vi "BigMAQ.vi"() -> ()   [LabVIEW 2019]
panel:
  out "Array 7":dbl[](array[numeric])
  out "Array 6":dbl[](array[numeric])
  out "Array 5":dbl[](array[numeric])
  out "Array 4":dbl[](array[numeric])
  out "Array 3":dbl[](array[numeric])
  out "Array 2":dbl[](array[numeric])
  out "x+y 2":dbl[](array[numeric])
  out "x+y":dbl[](array[numeric])
  out "Array":bool[](array[boolean])
  in  "IDs":T1
  out "Names":string[](array[string])
  in  "Status State":string="UI: Status"
  in  "Status":string
  out "States Out 2":string
  out "States Out":string
  out "Current State 2":string
  out "Arguments":string
  out "Current State":string
  out "Numeric 2":dbl
  out "Numeric":dbl
  in  "Image Data Range":cluster{dbl, dbl}(slide)={100.0, 0.0} scale=0.0..100.0
  out "SVG Object":T2
  in  "Name":string
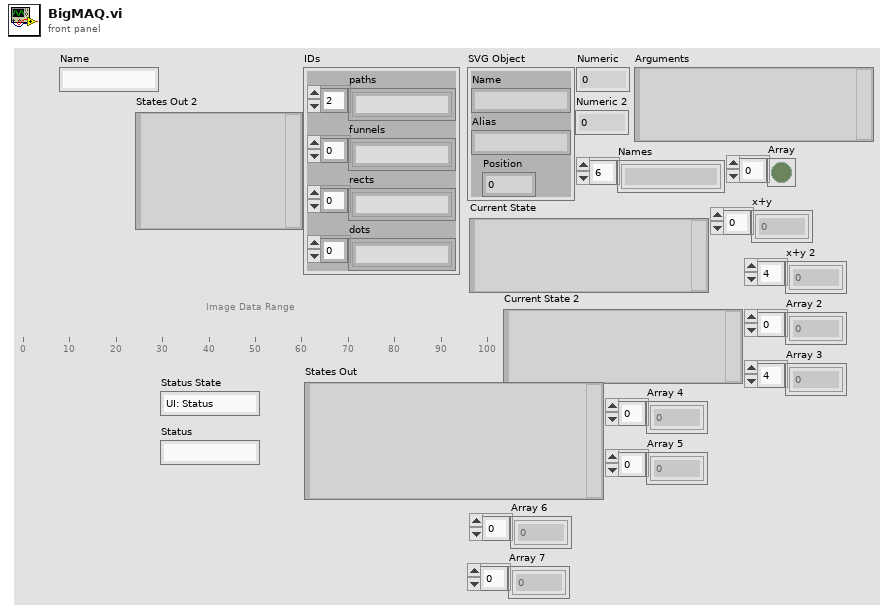
[diagram p1: front panel]
types:
  T1 = cluster{"paths":string[], "funnels":string[], "rects":string[], "dots":string[]}
  T2 = cluster{"Name":string, "Alias":string, "Position":i32}
  T3 = cluster{"Name":string, "Alias":string, "Position":i32}[]
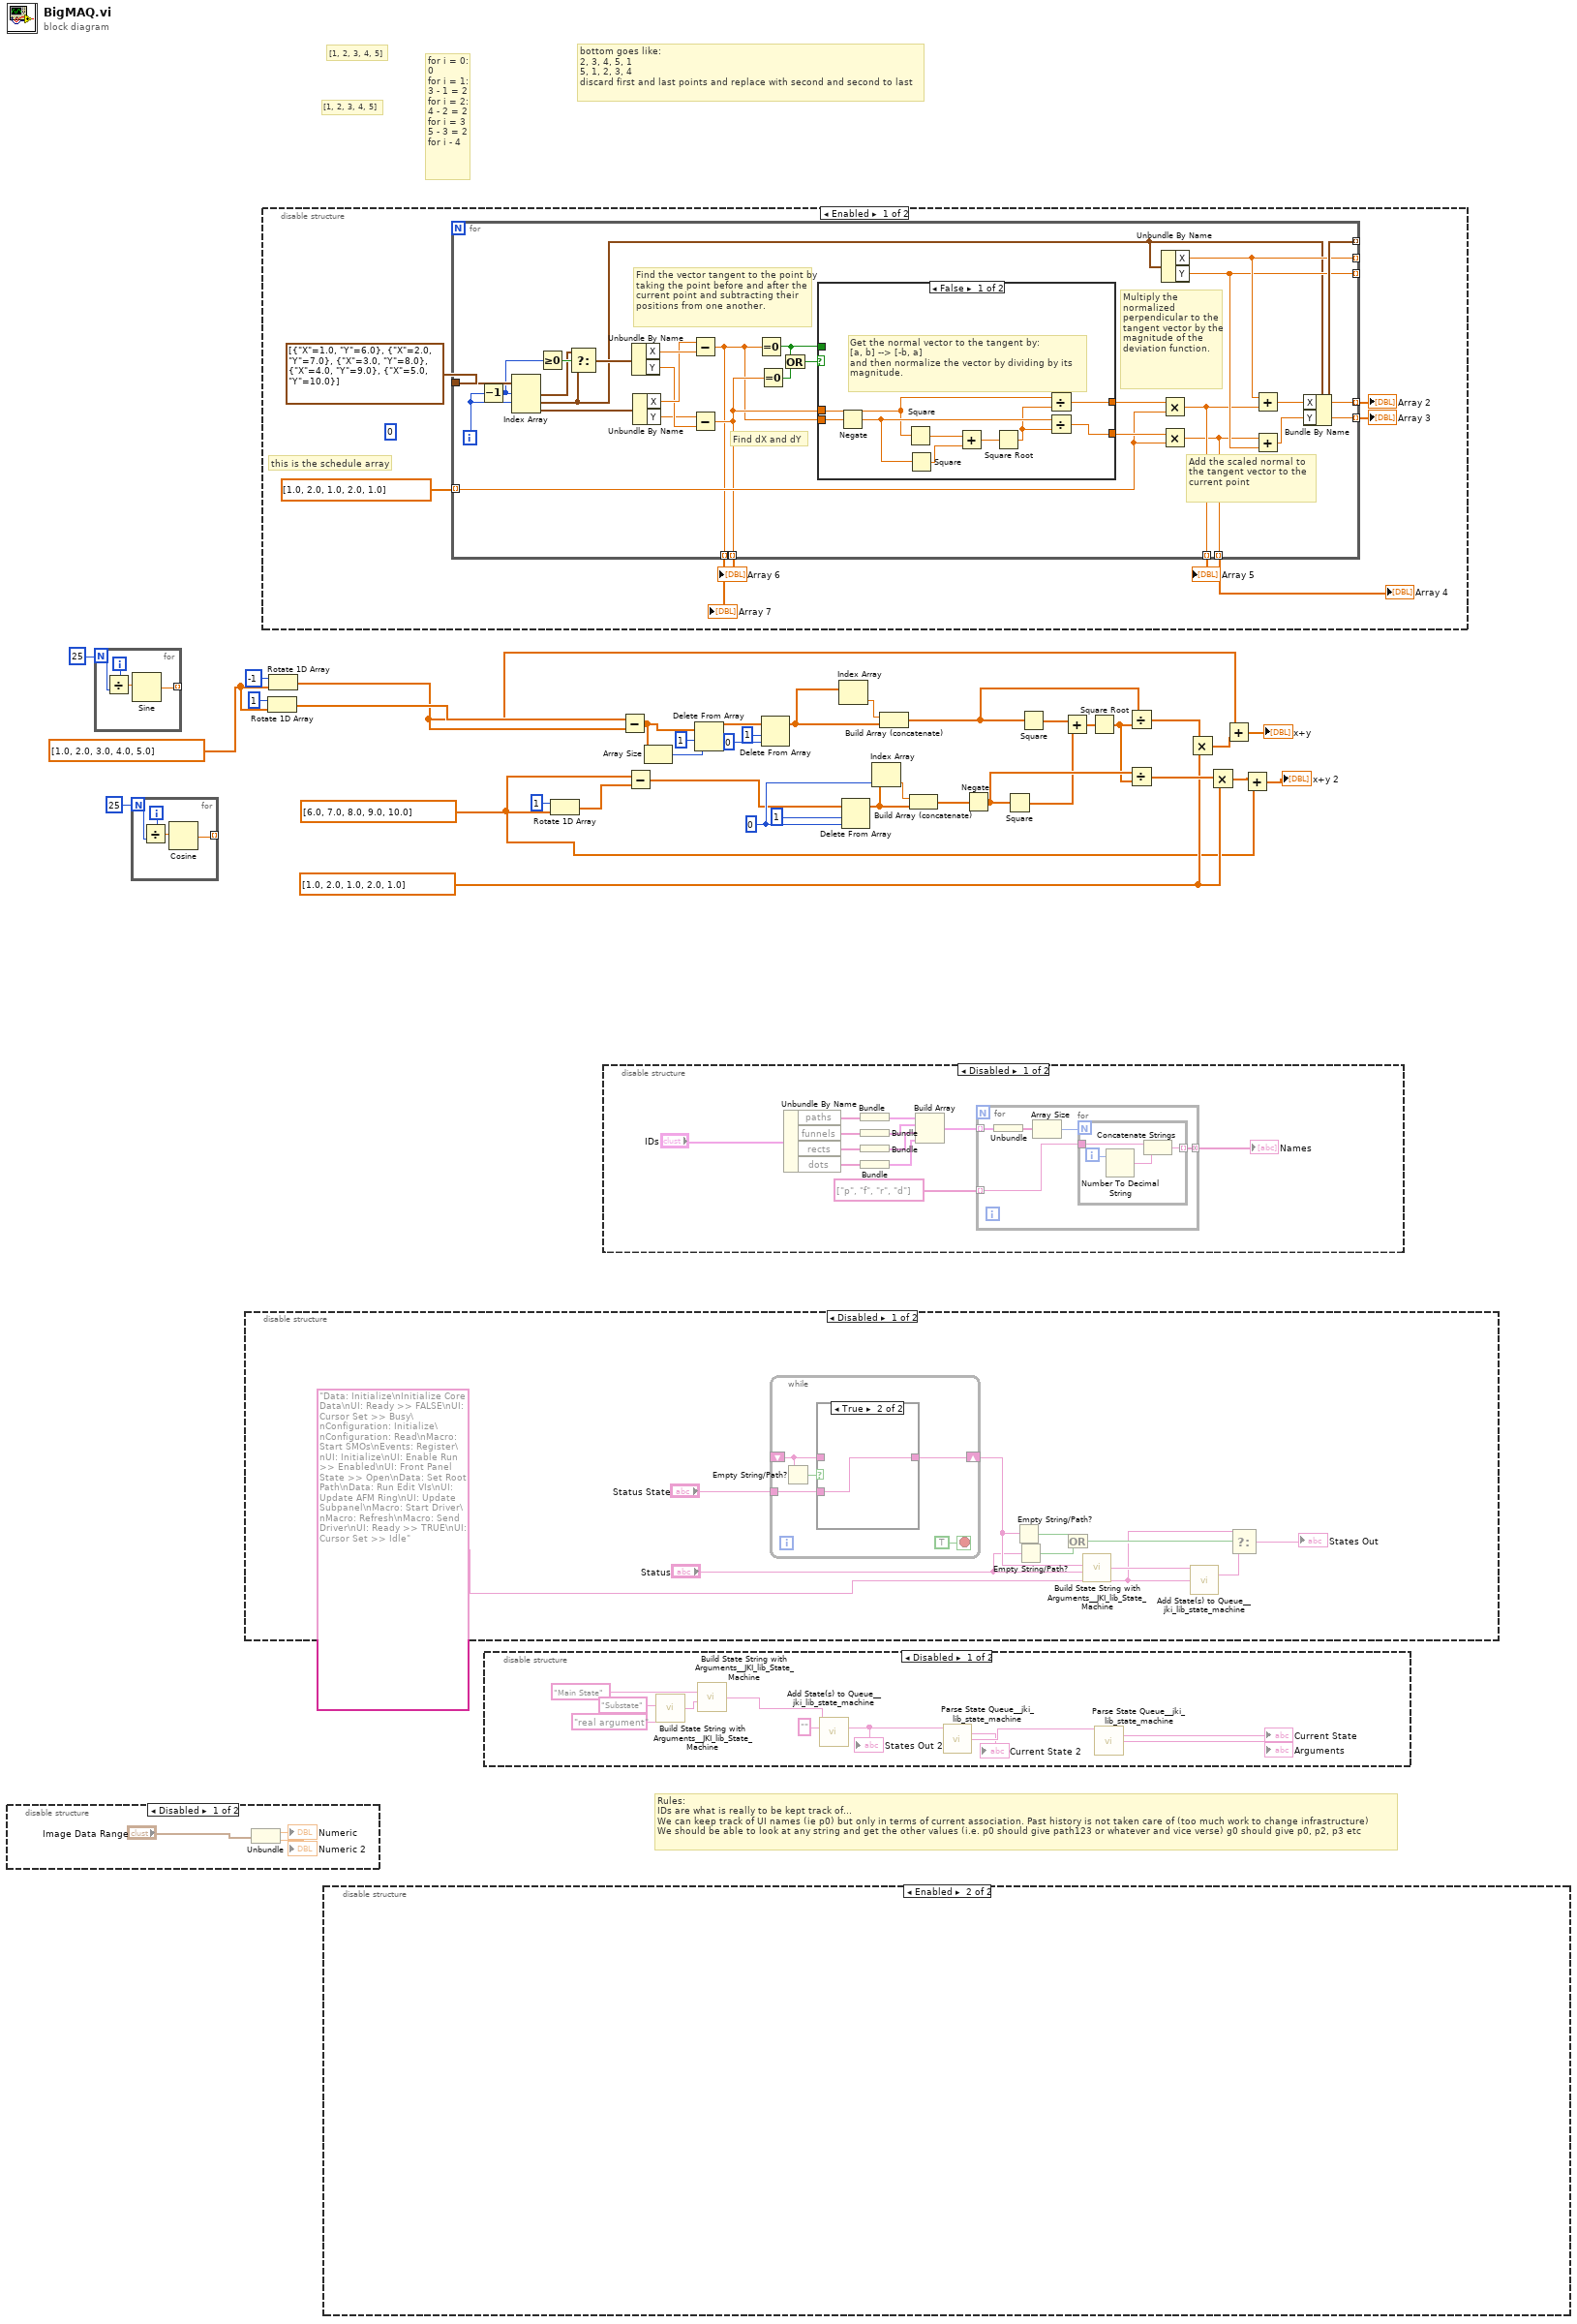
[diagram p0: block diagram]
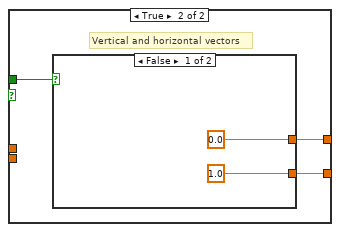
[diagram p7: hidden frame]
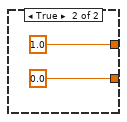
[diagram p8: hidden frame]
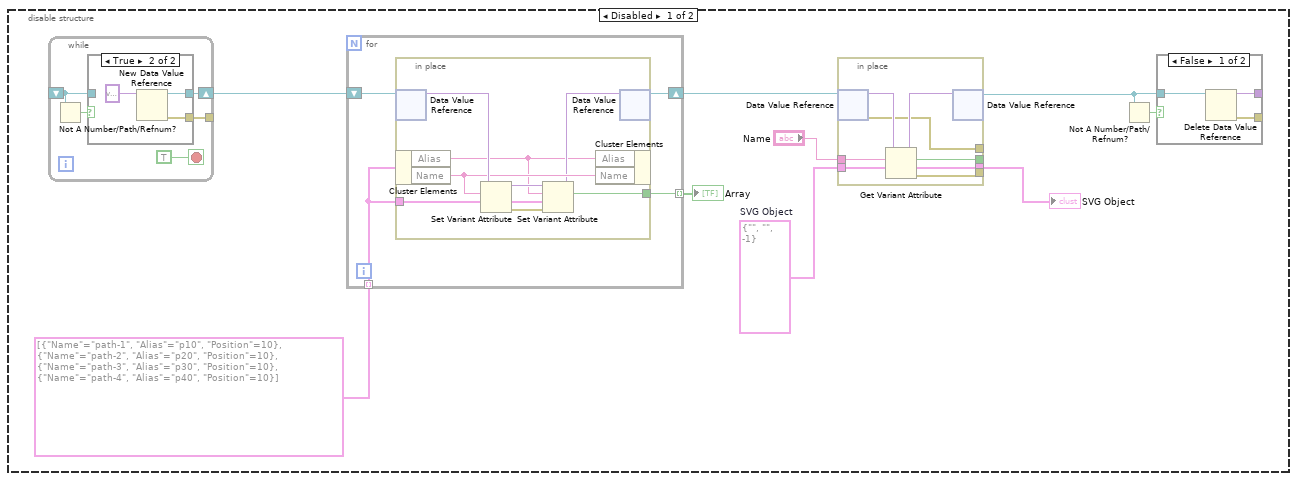
[diagram p10: hidden frame]
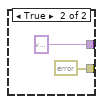
[diagram p11: hidden frame]
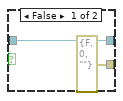
[diagram p12: hidden frame]
diagram:
  w7 = dbl[] [1.0, 2.0, 3.0, 4.0, 5.0] ("array")
  w20 = dbl[] [1.0, 2.0, 1.0, 2.0, 1.0] ("array")
  w31 = 0 ("index")
  w12 = dbl[] [6.0, 7.0, 8.0, 9.0, 10.0] ("array")
  # "bottom goes like:\n2, 3, 4, 5, 1\n5, 1, 2, 3, 4\ndiscard first and last points and replace with second and second to last"
  # "for i = 0:\n0\nfor i = 1:\n3 - 1 = 2\nfor i = 2:\n4 - 2 = 2\nfor i = 3 \n5 - 3 = 2\nfor i - 4"
  # "[1, 2, 3, 4, 5]"
  # "[1, 2, 3, 4, 5]"
  # "Rules:\nIDs are what is really to be kept track of... \nWe can keep track of UI names (ie p0) but only in terms of current association. Past history is not taken care of (too much work to change infrastructure)\nWe should be able to look at any string and get the other values (i.e. p0 should give path123 or whatever and vice verse) g0 should give p0, p2, p3 etc"
  n1 = disable-structure shown="Disabled" {
    frame Disabled {
      n2 = Unbundle("Image Data Range") -> (→"Numeric":dbl, →"Numeric 2":dbl)
    }
    frame Enabled {
    }
  }
  n3 = for {
    N: 25 -> [w43]
    tunnel: [w41] -> _ mode=indexing
    i -> [w44]
    n4 = Divide(x=w44, y=w43) -> (x/y=w42:dbl)
    n5 = Sine(x=w42) -> (sin(x)=w41:dbl)
  }
  n6 = for {
    N: 25 -> [w47]
    tunnel: [w45] -> _ mode=indexing
    i -> [w48]
    n7 = Divide(x=w48, y=w47) -> (x/y=w46:dbl)
    n8 = Cosine(x=w46) -> (cos(x)=w45:dbl)
  }
  n9 = disable-structure shown="Disabled" {
    frame Disabled {
      w49 = "Data: Initialize\nInitialize Core Data\nUI: Ready >> FALSE\nUI: Cursor Set >> Busy\nConfiguration: Initialize\nConfiguration: Read\nMacro: Start SMOs\nEvents: Register\nUI: Initialize\nUI: Enable Run >> Enabled\nUI: Front Panel State >> Open\nData: Set Root Path\nData: Run Edit VIs\nUI: Update AFM Ring\nUI: Update Subpanel\nMacro: Start Driver\nMacro: Refresh\nMacro: Send Driver\nUI: Ready >> TRUE\nUI: Cursor Set >> Idle"
      n10 = while {
        tunnel: "Status State" -> [w61]
        shift-right: [w62] -> w56
        shift-left: _ -> [w59]
        stop <- TRUE stop-if-true
        n11 = Empty String/Path?(string/path=w59) -> (empty?=w60:bool)
        n12 = case shown="True" w60 {
          tunnel: [w64 w65] -> w62
          tunnel: w61 -> [_ w65]
          tunnel: w59 -> [w64 _]
          frame False {
          }
          frame True {
          }
        }
      }
      n13 = Empty String/Path?(string/path=w56) -> (empty?=w54:bool)
      n14 = Empty String/Path?(string/path="Status") -> (empty?=w53:bool)
      n15 = Or(x=w54, y=w53) -> (x .or. y?=w52:bool)
      n16 = call <vilib>:"Build State String with Arguments__JKI_lib_State_Machine.vi"("Arguments (\"\")"="Status", "State"=w56) -> ("State with Arguments"=w57:string)  [unwired: 4 in]
      n17 = call <vilib>:"Add State(s) to Queue__jki_lib_state_machine.vi"("State(s) in Front (\"\")"=w57, "State(s) at Back (\"\")"=w49) -> ("States Out"=w51:string)  [unwired: 13 in]
      n18 = Select(t=w49, s=w52, f=w51) -> (s? t:f=→"States Out":string)
    }
    frame Enabled {
    }
  }
  n19 = disable-structure shown="Enabled" {
    frame Enabled {
      (unwired) 0
      # "this is the schedule array"
      n20 = for {
        tunnel: cluster{"X":dbl, "Y":dbl}[] [{"X"=1.0, "Y"=6.0}, {"X"=2.0, "Y"=7.0}, {"X"=3.0, "Y"=8.0}, {"X"=4.0, "Y"=9.0}, {"X"=5.0, "Y"=10.0}] ("array of clusters") -> [w100]
        tunnel: dbl[] [1.0, 2.0, 1.0, 2.0, 1.0] ("Y Values") -> [w88] mode=indexing
        tunnel: [w87] -> _ mode=indexing
        tunnel: [w78] -> w70 mode=indexing
        tunnel: [w86] -> w71 mode=indexing
        tunnel: [w85] -> _ mode=indexing
        tunnel: [w84] -> _ mode=indexing
        tunnel: [w77] -> w68 mode=indexing
        tunnel: [w76] -> w69 mode=indexing
        tunnel: [w75] -> w67 mode=indexing
        tunnel: [w74] -> w66 mode=indexing
        i -> [w91]
        # "Add the scaled normal to the tangent vector to the current point"
        # "Multiply the normalized perpendicular to the tangent vector by the magnitude of the deviation function."
        # "Find the vector tangent to the point by taking the point before and after the current point and subtracting their positions from one another."
        # "Find dX and dY"
        n21 = Decrement(x=w91) -> (x-1=w83:i32)
        n22 = Index Array(array=w100, index #1=w83, index #2=w91) -> (element #1=w79:cluster{"X":dbl, "Y":dbl}, element #2=w80:cluster{"X":dbl, "Y":dbl}, element #3=w99:cluster{"X":dbl, "Y":dbl})  [unwired: 1 in]
        n23 = Greater Or Equal To 0?(x=w83) -> (x >= 0?=w82:bool)
        n24 = Select(t=w79, s=w82, f=w80) -> (s? t:f=w81:cluster{"X":dbl, "Y":dbl})
        n25 = Unbundle By Name(w81) -> ("X"=w98:dbl, "Y"=w96:dbl)
        n26 = Unbundle By Name(w99) -> ("X"=w97:dbl, "Y"=w95:dbl)
        n27 = Subtract(x=w97, y=w98) -> (x-y=w74:dbl)
        n28 = Subtract(x=w95, y=w96) -> (x-y=w75:dbl)
        n29 = Equal To 0?(x=w74) -> (x = 0?=w92:bool)
        n30 = Equal To 0?(x=w75) -> (x = 0?=w93:bool)
        n31 = Or(x=w92, y=w93) -> (x .or. y?=w94:bool)
        n32 = case shown="False" w94 {
          tunnel: [w102 w110] -> w89
          tunnel: [w108 w111] -> w90
          tunnel: w74 -> [w109 _]
          tunnel: w75 -> [w101 _]
          tunnel: w92 -> [_ w112]
          frame False {
            # "Get the normal vector to the tangent by:\n[a, b] --> [-b, a]\nand then normalize the vector by dividing by its magnitude."
            n33 = Negate(x=w109) -> (-x=w104:dbl)
            n34 = Square(x=w101) -> (x^2=w107:dbl)
            n35 = Square(x=w104) -> (x^2=w106:dbl)
            n36 = Add(x=w107, y=w106) -> (x+y=w105:dbl)
            n37 = Square Root(x=w105) -> (sqrt(x)=w103:dbl)
            n38 = Divide(x=w101, y=w103) -> (x/y=w108:dbl)
            n39 = Divide(x=w104, y=w103) -> (x/y=w102:dbl)
          }
          frame True {
            # "Vertical and horizontal vectors"
            n40 = case shown="False" w112 {
              tunnel: [0.0 1.0] -> w111
              tunnel: [1.0 0.0] -> w110
              frame False {
              }
              frame True {
              }
            }
          }
        }
        n41 = Multiply(x=w90, y=w88) -> (x*y=w77:dbl)
        n42 = Multiply(x=w89, y=w88) -> (x*y=w76:dbl)
        n43 = Unbundle By Name(w80) -> ("X"=w85:dbl, "Y"=w84:dbl)
        n44 = Add(x=w85, y=w77) -> (x+y=w86:dbl)
        n45 = Add(x=w76, y=w84) -> (x+y=w78:dbl)
        n46 = Bundle By Name(cluster=w80, "X"=w86, "Y"=w78) -> (w87:cluster{"X":dbl, "Y":dbl})
      }
      "Array 2" <- w71
      "Array 3" <- w70
      "Array 4" <- w69
      "Array 5" <- w68
      "Array 6" <- w67
      "Array 7" <- w66
    }
    frame Disabled {
    }
  }
  n47 = Rotate 1D Array(1:w7, 2:1 ("n")) -> (0:w6:dbl[])
  n48 = Rotate 1D Array(1:w7, 2:-1 ("n")) -> (0:w5:dbl[])
  n49 = disable-structure shown="Enabled" {
    frame Disabled {
      w122 = T2 {"Name"="", "Alias"="", "Position"=-1}  # SVG Object
      n50 = while {
        shift-right: [w154] -> w121
        shift-left: _ -> [w152]
        tunnel: [w151] -> _
        stop <- TRUE stop-if-true
        n51 = Not A Number/Path/Refnum?(number/path/refnum=w152) -> (NaN/Path/Refnum?=w155:bool)
        n52 = case shown="True" w155 {
          tunnel: w152 -> [w157 _]
          tunnel: [w157 w159] -> w154
          tunnel: [errorcluster {"status"=FALSE, "code"=0, "source"=""} ("error out") w158] -> w151
          frame False {
          }
          frame True {
            n53 = New Data Value Reference(data value=variant) -> (data value reference=w159:refnum<data-value>, error out=w158:errorcluster)  [unwired: 1 in]
          }
        }
      }
      n54 = for {
        tunnel: T3 [{"Name"="path-1", "Alias"="p10", "Position"=10}, {"Name"="path-2", "Alias"="p20", "Position"=10}, {"Name"="path-3", "Alias"="p30", "Position"=10}, {"Name"="path-4", "Alias"="p40", "Position"=10}] -> [w127] mode=indexing
        shift-right: [w128] -> w120
        shift-left: w121 -> [w129]
        tunnel: [w126] -> w117 mode=indexing
        n55 = in-place {
          in-place-border: w127 -> [w131]
          in-place-border: [w130] -> w126
          n56 = in-place-dvr #1(w129) -> (w137:variant)  [unwired: 1 out]
          n57 = in-place-cluster #2(w127) -> ("Alias"=w132:string, "Name"=w136:string)
          n58 = Set Variant Attribute(Variant=w137, name=w136, value=w131) -> (Variant out=w134:variant, error out=w135:errorcluster)  [unwired: 1 in, 1 out]
          n59 = Set Variant Attribute(Variant=w134, name=w132, value=w131, error in=w135) -> (Variant out=w133:variant, replaced=w130:bool)  [unwired: 1 out]
          n60 = in-place-cluster #2("Alias"=w132, "Name"=w136) -> ()  [unwired: 1 out]
          n61 = in-place-dvr #1(w133) -> (w128:refnum<data-value>)  [unwired: 1 out]
        }
      }
      "Array" <- w117
      n62 = in-place {
        in-place-border: [w150] -> w119
        in-place-border: "Name" -> [w147]
        in-place-border: w122 -> [w146]
        in-place-border: [w145] -> _
        in-place-border: [w144] -> _
        in-place-border: [w143] -> _
        n63 = in-place-dvr #3(w120) -> (w149:variant, w144:errorcluster)
        n64 = Get Variant Attribute(Variant=w149, name=w147, default value (empty Variant)=w146) -> (duplicate Variant=w148:variant, found=w145:bool, value=w150:T2, error out=w143:errorcluster)  [unwired: 1 in]
        n65 = in-place-dvr #3(w148) -> (w123:refnum<data-value>)  [unwired: 1 out]
      }
      "SVG Object" <- w119
      n66 = Not A Number/Path/Refnum?(number/path/refnum=w123) -> (NaN/Path/Refnum?=w124:bool)
      n67 = case shown="False" w124 {
        tunnel: w123 -> [w140 _]
        tunnel: [w138 errorcluster {"status"=FALSE, "code"=0, "source"=""} ("error out")] -> _
        tunnel: [w139 variant] -> _
        frame False {
          n68 = Delete Data Value Reference(data value reference=w140) -> (data value=w139:variant, error out=w138:errorcluster)  [unwired: 1 in]
        }
        frame True {
        }
      }
    }
    frame Enabled {
    }
  }
  n69 = disable-structure shown="Disabled" {
    frame Disabled {
      n70 = call <vilib>:"Build State String with Arguments__JKI_lib_State_Machine.vi"("Arguments (\"\")"="real argument" ("Arguments (\"\")"), "State"="Substate") -> ("State with Arguments"=w167:string)  [unwired: 4 in]
      n71 = call <vilib>:"Build State String with Arguments__JKI_lib_State_Machine.vi"("Arguments (\"\")"=w167, "State"="Main State") -> ("State with Arguments"=w164:string)  [unwired: 4 in]
      n72 = call <vilib>:"Add State(s) to Queue__jki_lib_state_machine.vi"("State(s) in Front (\"\")"=w164, "State(s) in (\"\")"="" ("State(s) in (\"\")")) -> ("States Out"=w171:string)  [unwired: 13 in]
      "States Out 2" <- w171
      n73 = call <vilib>:"Parse State Queue__jki_lib_state_machine.vi"("State Queue"=w171) -> ("Current State"=→"Current State 2":string, "Arguments"=w162:string)  [unwired: 12 in, 1 out]
      n74 = call <vilib>:"Parse State Queue__jki_lib_state_machine.vi"("State Queue"=w162) -> ("Current State"=→"Current State":string, "Arguments"=→"Arguments":string)  [unwired: 12 in, 1 out]
    }
    frame Enabled {
    }
  }
  n75 = Rotate 1D Array(1:w12, 2:1 ("n")) -> (0:w36:dbl[])
  n76 = disable-structure shown="Disabled" {
    frame Disabled {
      n77 = Unbundle By Name("IDs") -> ("paths"=w182:string[], "funnels"=w181:string[], "rects"=w180:string[], "dots"=w179:string[])
      n78 = Bundle("paths"=w182) -> (w178:cluster{"paths":string[]})  [unwired: 1 in]
      n79 = Bundle("funnels"=w181) -> (w177:cluster{"funnels":string[]})  [unwired: 1 in]
      n80 = Bundle("rects"=w180) -> (w176:cluster{"rects":string[]})  [unwired: 1 in]
      n81 = Bundle("dots"=w179) -> (w175:cluster{"dots":string[]})  [unwired: 1 in]
      n82 = Build Array(w178, w177, w176, w175) -> (w173:cluster{"dots":string[]}[])
      n83 = for {
        tunnel: string[] ["p", "f", "r", "d"] -> [w185] mode=indexing
        tunnel: w173 -> [w188] mode=indexing
        tunnel: [w184] -> w172 mode=concatenating
        n84 = Unbundle(w188) -> ("dots"=w187:string[])
        n85 = Array Size(array=w187) -> (size(s)=w186:i32)
        n86 = for {
          N: w186 -> [_]
          tunnel: w185 -> [w191]
          tunnel: [w189] -> w184 mode=indexing
          i -> [w192]
          n87 = Number To Decimal String(number=w192) -> (decimal integer string=w190:string)  [unwired: 1 in]
          n88 = Concatenate Strings(w191, w190) -> (w189:string)
        }
      }
      "Names" <- w172
    }
    frame Enabled {
    }
  }
  n89 = Subtract(x=w6, y=w5) -> (x-y=w2:dbl[])
  n90 = Subtract(x=w12, y=w36) -> (x-y=w29:dbl[])
  n91 = Array Size(array=w2) -> (size(s)=w1:i32)
  n92 = Delete From Array(array=w2, length=1, index=w1) -> (array with subset deleted=w4:dbl[])  [unwired: 1 out]
  n93 = Delete From Array(array=w4, length=1, index=0) -> (array with subset deleted=w15:dbl[])  [unwired: 1 out]
  n94 = Index Array(array=w15) -> (element=w33:dbl)  [unwired: 1 in]
  n95 = Delete From Array(array=w29, length=1, index=w31) -> (array with subset deleted=w14:dbl[])  [unwired: 1 out]
  n96 = Index Array(array=w14, index=w31) -> (element=w32:dbl)
  n97 = Build Array (concatenate)(w33, w15) -> (w25:dbl[])
  n98 = Build Array (concatenate)(w32, w14) -> (w28:dbl[])
  n99 = Negate(x=w28) -> (-x=w24:dbl[])
  n100 = Square(x=w24) -> (x^2=w23:dbl[])
  n101 = Square(x=w25) -> (x^2=w27:dbl[])
  n102 = Add(x=w27, y=w23) -> (x+y=w26:dbl[])
  n103 = Square Root(x=w26) -> (sqrt(x)=w13:dbl[])
  n104 = Divide(x=w25, y=w13) -> (x/y=w22:dbl[])
  n105 = Divide(x=w24, y=w13) -> (x/y=w21:dbl[])
  n106 = Multiply(x=w22, y=w20) -> (x*y=w19:dbl[])
  n107 = Multiply(x=w21, y=w20) -> (x*y=w18:dbl[])
  n108 = Add(x=w5, y=w19) -> (x+y=→"x+y":dbl[])
  n109 = Add(x=w18, y=w12) -> (x+y=→"x+y 2":dbl[])
